vi "Convertor.vi"(11 "格式化机器人指令":string[][](array[string])) -> (1 "机器人对话指令数据簇数组(Dialogue)":T2(array[cluster]), 2 "机器人语音指令数据簇数组(Voice)":T1(array[cluster]), 3 "命令个数":i32)   [LabVIEW 2014, in "Dialogue.lvlib" / "Dialogue.lvclass"]
uses:
  Dialogue.lvclass
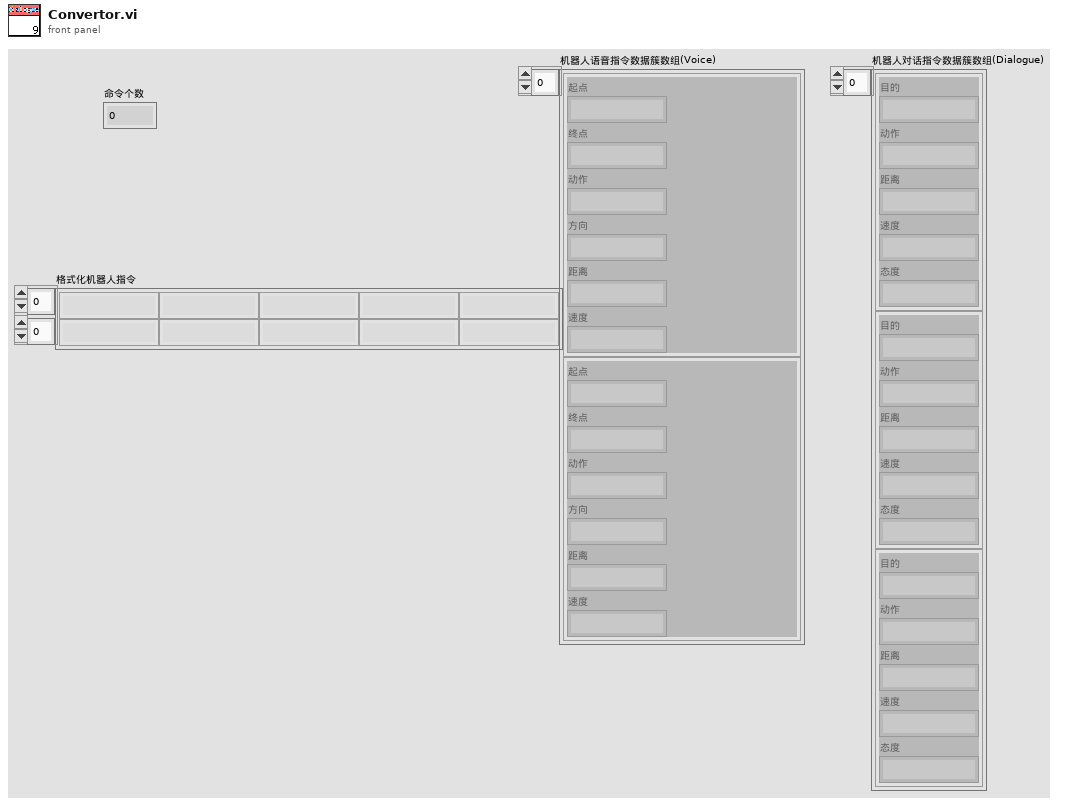
[diagram p1: front panel]
types:
  T1 = cluster{"起点":string, "终点":string, "动作":string, "方向":string, "距离":string, "速度":string}[]
  T2 = cluster{"目的":string, "动作":string, "距离":string, "速度":string, "态度":string}[]
  T3 = cluster{"起点":string, "终点":string, "动作":string, "方向":string, "距离":string, "速度":string}
  T4 = cluster{"目的":string, "动作":string, "距离":string, "速度":string, "态度":string}
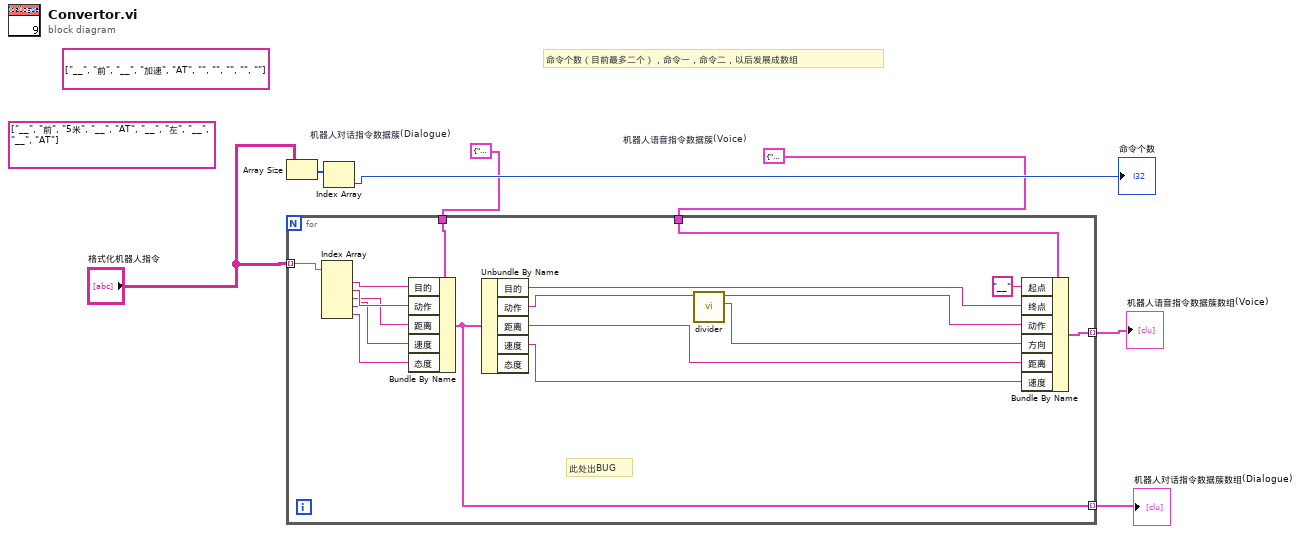
[diagram p0: block diagram]
diagram:
  w3 = T3 {"起点"="", "终点"="", "动作"="", "方向"="", "距离"="", "速度"=""}  # 机器人语音指令数据簇(Voice)
  w5 = T4 {"目的"="", "动作"="", "距离"="", "速度"="", "态度"=""}  # 机器人对话指令数据簇(Dialogue)
  (unwired) string[][] [["__", "前", "__", "加速", "AT"], ["", "", "", "", ""]] ("格式化机器人指令 2")
  (unwired) string[][] [["__", "前", "5米", "__", "AT"], ["__", "左", "__", "__", "AT"]] ("格式化机器人指令 2")
  # "命令个数（目前最多二个），命令一，命令二，以后发展成数组"
  n1 = Array Size(array="格式化机器人指令") -> (size(s)=w7:i32[])
  n2 = for {
    tunnel: "格式化机器人指令" -> [w23] mode=indexing
    tunnel: w5 -> [w24]
    tunnel: [w16] -> w4 mode=indexing
    tunnel: w3 -> [w17]
    tunnel: [w11] -> w2 mode=indexing
    # "此处出BUG"
    n3 = Index Array(array=w23) -> (element #1=w22:string, element #2=w21:string, element #3=w20:string, element #4=w19:string, element #5=w18:string)  [unwired: 5 in]
    n4 = Bundle By Name(cluster=w24, "目的"=w22, "动作"=w21, "距离"=w20, "速度"=w19, "态度"=w18) -> (w16:T4)
    n5 = Unbundle By Name(w16) -> ("目的"=w15:string, "动作"=w10:string, "距离"=w13:string, "速度"=w14:string)  [unwired: 1 out]
    n6 = call "divider.vi"("动作"=w10) -> ("方向"=w8:string, "动作 out"=w9:string)  [unwired: 9 in]
    n7 = Bundle By Name(cluster=w17, "起点"="__", "终点"=w15, "动作"=w9, "方向"=w8, "距离"=w13, "速度"=w14) -> (w11:T3)
  }
  "机器人对话指令数据簇数组(Dialogue)" <- w4
  "机器人语音指令数据簇数组(Voice)" <- w2
  n8 = Index Array(array=w7) -> (element=→"命令个数":i32)  [unwired: 1 in]
